vi "Edit Line.vi"(8 "error in":errorcluster, 10 "Line Name":string, 11 "References":T1) -> (0 "error out":errorcluster, 2 "change?":bool)   [LabVIEW 2015, in "Scan Engine editor node.lvclass"]
doc: "This VI edits the properties of a line. It will unlick channels and tags and create new links to channels and tags."
uses:
  Scan Engine editor node.lvclass
  <vilib>/NI/DCAF/Tag Editor Core/Table API/Table Manager/object ref.ctl
  <vilib>/NI/DCAF/Tag Editor Core/Configuration Editor/Classes/Engine Parent/Engine Parent Editor Node.lvclass
  <vilib>/NI/DCAF/Tag Editor Core/Configuration Editor/Classes/Module editor node/module editor node.lvclass
  configuration/Scan Engine configuration.lvclass
  configuration/Scan Engine configuration.lvclass/Scan Engine configuration.ctl
  <vilib>/NI/Configuration Framework/serializable configuration/NISE_CEF_serializable configuration.lvclass/NISE_CEF_serializable configuration.ctl
  <vilib>/Utility/LVClass/Get LV Class Name.vi
  <vilib>/NI/Configuration Framework/error generator/NISE_error generator.vi
  <vilib>/NI/Tag Bus Module Framework/channel/TBM channel.lvclass
  <vilib>/NI/Configuration Framework/serializable configuration/NISE_CEF_serializable configuration.lvclass
  <vilib>/NI/DCAF/Tag Editor Core/Table API/Table Manager/Table Manager.lvclass
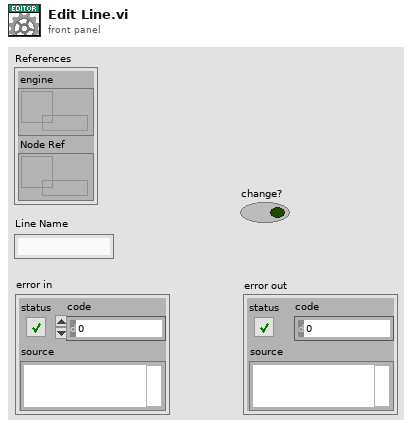
[diagram p1: front panel]
types:
  T1 = typedef "Table Manager.lvlib/Table Manager.lvclass/object ref.ctl" = cluster{"engine":refnum<data-value>, "Node Ref":refnum<data-value>}
  T2 = typedef "Scan Engine configuration.lvclass/Line.ctl" = cluster{"channel":refnum<class "TBM channel.lvclass">, "Tag":string}
  T3 = typedef "Scan Engine editor node.lvclass/Mappings.ctl" = cluster{"Line":T2, "Maps":T4[]}
  T4 = typedef "Scan Engine editor node.lvclass/Map.ctl" = cluster{"channel":refnum<class "TBM channel.lvclass">, "tag name":string}
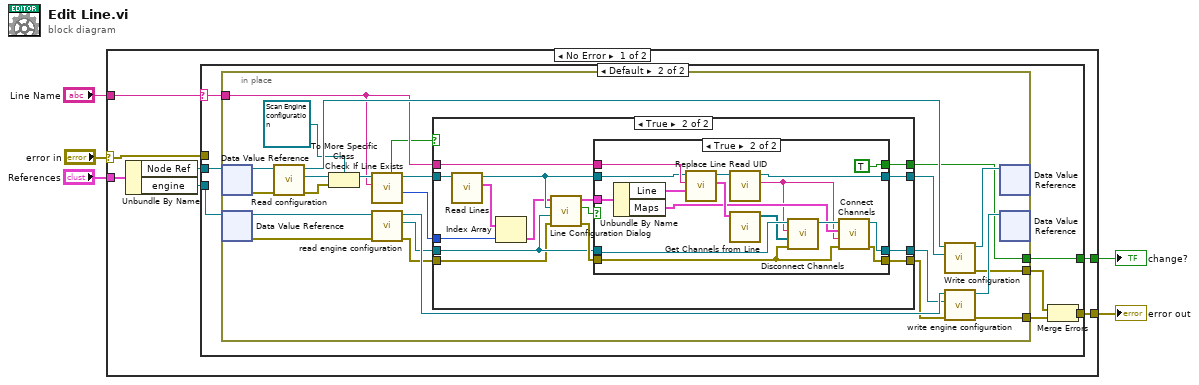
[diagram p0: block diagram]
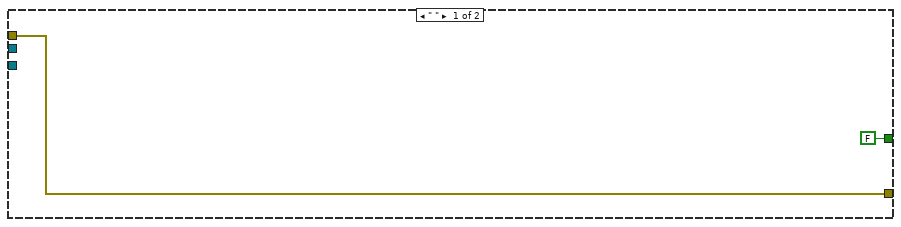
[diagram p2: hidden frame]
diagram:
  n1 = case shown="No Error" "error in" {
    selector: "error in" -> [w6 w83]
    tunnel: "References" -> [w10 _]
    tunnel: "Line Name" -> [w7 _]
    tunnel: [w9 w83] -> w2
    tunnel: [w8 _] -> w1
    frame No Error {
      n2 = Unbundle By Name(w10) -> ("Node Ref"=w12:refnum<data-value>, "engine"=w11:refnum<data-value>)
      n3 = case shown="Default" w7 {
        selector: w7 -> [_ w15]
        tunnel: w12 -> [_ w21]
        tunnel: w11 -> [_ w20]
        tunnel: [w13 w17] -> w9
        tunnel: [FALSE ("change?") w16] -> w8
        tunnel: w6 -> [w13 _]
        frame " " {
        }
        frame Default {
          n4 = in-place {
            in-place-border: [w27] -> w19
            in-place-border: [w42] -> w18
            in-place-border: [w26] -> w16
            in-place-border: w15 -> [w32]
            n5 = in-place-dvr #1(w21) -> (w39:refnum<class "module editor node.lvclass">, w33:errorcluster)
            n6 = in-place-dvr #2(w20) -> (w45:refnum<class "Engine Parent Editor Node.lvclass">, w44:errorcluster)
            n7 = call-dynamic "Read configuration.vi"("error in"=w33, "NISE_CEF_serializable node in"=w39) -> ("error out"=w36:errorcluster, "configuration"=w37:refnum<class "NISE_CEF_serializable configuration.lvclass">, "NISE_CEF_serializable node out"=w38:refnum<class "module editor node.lvclass">)  [unwired: 7 in]
            n8 = To More Specific Class(target class=refnum<class "Scan Engine configuration.lvclass"> refnum ("tag bus configurable plugin module configuration"), reference=w37, error in=w36) -> (specific class reference=w34:refnum<class "Scan Engine configuration.lvclass">)  [unwired: 1 out]
            n9 = call-dynamic "Check If Line Exists.vi"("name to locate"=w32, "Scan Engine configuration in"=w34) -> ("index"=w29:i32, "Scan Engine configuration out"=w30:refnum<class "Scan Engine configuration.lvclass">, "found?"=w24:bool)  [unwired: 5 in, 2 out]
            n10 = call <vilib>:"read engine configuration.vi"("error in"=w44, "Engine Parent Editor Node in"=w45) -> ("error out"=w23:errorcluster, "engine configuration"=w28:refnum<class "engine configuration.lvclass">, "Engine Parent Editor Node out"=w41:refnum<class "Engine Parent Editor Node.lvclass">)  [unwired: 7 in]
            n11 = case shown="True" w24 {
              tunnel: w30 -> [w48 w61]
              tunnel: w28 -> [w47 w51]
              tunnel: w32 -> [_ w63]
              tunnel: [w48 w55] -> w31
              tunnel: w29 -> [_ w58]
              tunnel: [_ w53] -> w26
              tunnel: [w47 w52] -> w25
              tunnel: w23 -> [w46 w50]
              tunnel: [w46 w49] -> w22
              frame False {
              }
              frame True {
                n12 = call "Read Lines.vi"("Scan Engine configuration in"=w61) -> ("Lines"=w59:T2[], "Scan Engine configuration out"=w60:refnum<class "Scan Engine configuration.lvclass">)  [unwired: 8 in, 1 out]
                n13 = Index Array(array=w59, index=w58) -> (element=w57:T2)
                n14 = call "Line Configuration Dialog.vi"("error in"=w50, "engine configuration in"=w51, "tag bus configurable plugin module configuration"=w60, "Line"=w57) -> ("error out"=w62:errorcluster, "changed"=w54:bool, "Mappings out"=w56:T3)  [unwired: 4 in, 1 out]
                n15 = case shown="True" w54 {
                  tunnel: w63 -> [_ w82]
                  tunnel: w51 -> [w65 w81]
                  tunnel: w62 -> [w64 w68]
                  tunnel: w60 -> [w66 w77]
                  tunnel: w56 -> [_ w76]
                  tunnel: [w66 w74] -> w55
                  tunnel: [_ TRUE ("change?")] -> w53
                  tunnel: [w65 w69] -> w52
                  tunnel: [w64 w67] -> w49
                  frame False {
                  }
                  frame True {
                    n16 = Unbundle By Name(w76) -> ("Line"=w75:T2, "Maps"=w72:T4[])
                    n17 = call "Replace Line.vi"("New Line"=w75, "Line Name"=w82, "Scan Engine configuration in"=w77) -> ("Old Line"=w79:T2, "Scan Engine configuration out"=w80:refnum<class "Scan Engine configuration.lvclass">)  [unwired: 6 in, 1 out]
                    n18 = call <vilib>:"Read UID.vi"("configuration in"=w80) -> ("instance id"=w71:string, "configuration out"=w74:refnum<class "Scan Engine configuration.lvclass">)  [unwired: 8 in, 1 out]
                    n19 = call "Get Channels from Line.vi"("Line"=w79) -> ("Array"=w78:refnum<class "TBM channel.lvclass">[])  [unwired: 10 in]
                    n20 = call "Disconnect Channels.vi"("error in (no error)"=w68, "Deleted Channels"=w78, "instance id"=w71, "engine configuration in"=w81) -> ("engine configuration out"=w73:refnum<class "engine configuration.lvclass">)  [unwired: 6 in, 1 out]
                    n21 = call "Connect Channels.vi"("error in (no error)"=w68, "instance id"=w71, "Maps"=w72, "engine configuration in"=w73) -> ("error out"=w67:errorcluster, "engine configuration out"=w69:refnum<class "engine configuration.lvclass">)  [unwired: 6 in]
                  }
                }
              }
            }
            n22 = call-dynamic "Write configuration.vi"("configuration"=w31, "NISE_CEF_serializable node in"=w38) -> ("error out"=w27:errorcluster, "NISE_CEF_serializable node out"=w40:refnum<class "module editor node.lvclass">)  [unwired: 8 in]
            n23 = call <vilib>:"write engine configuration.vi"("error in"=w22, "engine configuration"=w25, "Engine Parent Editor Node in"=w41) -> ("error out"=w42:errorcluster, "Engine Parent Editor Node out"=w43:refnum<class "Engine Parent Editor Node.lvclass">)  [unwired: 7 in]
            n24 = in-place-dvr #1(w40) -> ()  [unwired: 2 out]
            n25 = in-place-dvr #2(w43) -> ()  [unwired: 2 out]
          }
          n26 = Merge Errors(w19, w18) -> (w17:errorcluster)
        }
      }
    }
    frame Error {
    }
  }
  "change?" <- w1
  "error out" <- w2
